vi "AlliGator Intensity Time Trace Panel.vi"() -> ()   [LabVIEW 2021, in "AlliGator Intensity Time Trace.lvlib"]
uses:
  AlliGator Intensity Time Trace.lvlib
  Globals, Variables, Constants/AlliGator Refnums List.ctl
  AlliGator Intensity Time Trace Ctrl Refnums.ctl
  Settings/AlliGator Settings List.ctl
  Action Engine/AlliGator Q Element.ctl
  Action Engine/AlliGator Q Event.ctl
  Graphs/XY Graph/XY Graph Event.ctl
  <vilib>/Utility/miscctls.llb/LVPoint32TypeDef.ctl
  Variant/Variant to Data/Variant to Boolean.vi
  Settings/AlliGator Settings+.lvlib
  Variant/Variant to Data/Variant to Data.lvlib
  Notebook/Notebook.lvlib
  Action Engine/AlliGator Action Engine.lvlib
  GUI/GUI.lvlib
  GUI/AlliGator GUI.lvlib
  Error/Error.lvlib
  Graphs/XY Graph/XY Graph Add-Ons.lvlib
  Python Plugins API/AlliGator Python Plugins.lvlib
  Decay Analysis/Decay Processing/AlliGator Decay Processing.lvlib
  Utilities/Utilities.lvlib
panel:
  in  "Use File Timestamp":bool=TRUE
  in  "Time Step":dbl[unit]=1.0 format="%#_5g"
  in  "Pin Button":bool=TRUE
  out "Intensity Time Trace TipStrip":string caption="Lifetime Graph TipStrip"
  out "Intensity Time Trace":cluster{"X Array":dbl[], "Y Array":dbl[]}[](graph)
  in  "Intensity Correction File":path
  in  "Use Intensity Correction File":bool
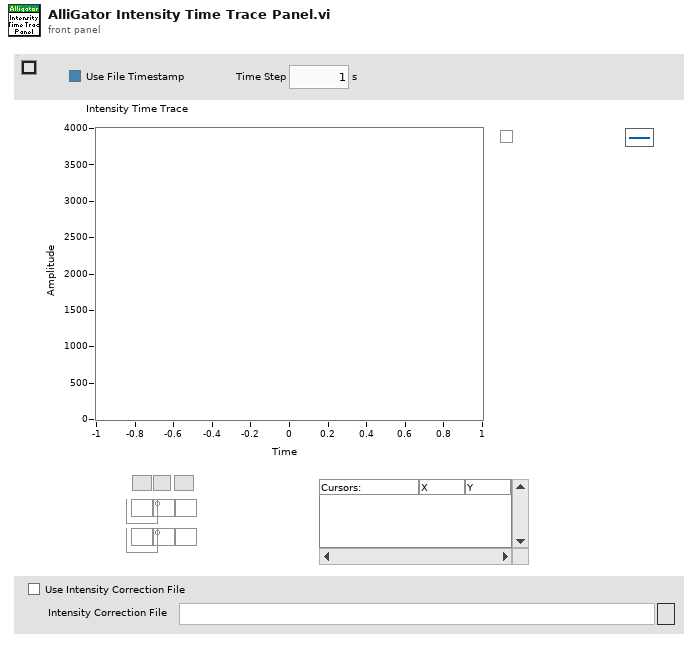
[diagram p1: front panel]
types:
  T1 = typedef "AlliGator Intensity Time Trace.lvlib/AlliGator Intensity Time Trace Ctrl Refnums.ctl" = cluster{"Intensity Time Trace":refnum<vi>, "Time Step":refnum<vi>, "Use File Timestamp":refnum<vi>}
  T2 = typedef "AlliGator GUI.lvlib/AlliGator Refnums List.ctl" = enum16{"---------- AlliGator Control Refnums ----------", "AlliGator Tab Control Refnum", "Dataset Ctrl Refnums", "Image Histogram Ctrl Refnums", "Intensity Time Trace Ctrl Refnums", "Decay Graph Ctrl Refnums", "Decay Statistics Graph Ctrl Refnums", "Phasor Graph Ctrl Refnums", "Phasor Ratio Graph Ctrl Refnums", "Phasor Plot Ctrl Refnums", "Lifetime & Other Parameters Ctrl Refnums", "Decay Fit Parameter Map Ctrl Refnums", "Parameter Map Ctrl Refnums", "Other AlliGator Ctrl Refnums", "---------- AlliGator Menu Refnums ----------", "AlliGator Menu", "---------- IO Device ID ----------", "Mouse ID", "Keyboard ID"}
  T3 = cluster{"Event Registration Refnum":refnum<event-registration>, "Event Registration Refnum":refnum<event-registration>}
  T4 = typedef "AlliGator Settings+.lvlib/AlliGator Settings List.ctl" = enum16{"GUI:Visible Settings Tab", "GUI:Last Run Version", "Source Image:Use Image Histogram for Contrast", "Source Image:Low Count Pixels Rejection Options", "Source Image:High Count Pixels Rejection Options", "Source Image:Use Image Brightness", "Source Image:Blend Overlay with Image Background", "Source Image:Use Fixed ROI Diameter", "Source Image:ROI Diameter", "Source Image:ROI Center Color", "Source Image:Peak Threshold", "Source Image:Intensity Threshold", "Source Image:Image Binning Options", "Source Image:Image Smoothing Options", "Source Image:Image Histogram Active", "Source Image:Invert Binary Mask", "Source Image:Hot Pixel Removal", "Source Image:Overlay Analyzed ROI Center", "Source Image:Auto-Adjust Contrast", "Source Image:Histogram Lower Percentile", "Source Image:Histogram Upper Percentile", "Source Image:Lock ROI with Maps", "Source Image:Save Source Image", "Source Image:Scale Bar Options", "Source Image:Image Resolution (Pixel Size)", "Source Image:Flatfield Correction", "Source Image:Show Dead Left Columns Correction", "Source Image:Dead Left Columns Correction", "Source Image:Image Pre-Processing Operations Order", "Source Image:Overlay ROI Median", "Source Image:Median Overlay Color", "Data Information:Gate Width", "Data Information:Nanotime Gate Separation", "Data Information:Macrotime Gate Separation", "Data Information:Gate Step", "Data Information:# Gates", "Data Information:Gate Image Exposure", "Data Information:Gate Image Integration", "Data Information:Gates to Skip", "Data Information:Gates to Keep", "Data Information:Define Gates to", "Data Information:Channel Name", "Data Information:Available Channel Names", "Data Information:Channel Arithmetic", "Data Information:Background File Subtraction", "Data Information:Background File", "Data Information:Background Scaling Factor", "Data Information:Background Pile-up Correction", "Data Information:Background Pixel Well Capacity", "Data Information:Laser Period", "Data Information:SYNC Period", "Data Information:Pile-up Correction", "Data Information:Pixel Well Capacity", "Data Information:Dataset Scaling Factor", "Fluorescence Decay_Decay Pre-Processing:Reverse Gates", "Fluorescence Decay_Decay Pre-Processing:Verbose Decay Pre-Processing", "Fluorescence Decay_Decay Pre-Processing:Use Decay Pre-Processing", "Fluorescence Decay_Decay Pre-Processing:Background Subtraction", "Fluorescence Decay_Decay Pre-Processing:Background Definition Range", "Fluorescence Decay_Decay Pre-Processing:Baseline Subtraction Method", "Fluorescence Decay_Decay Pre-Processing:Decay Pre-Processing Operations Order", "Fluorescence Decay_Decay Pre-Processing:Smoothing Parameter", "Fluorescence Decay_Decay Pre-Processing:Shift Decay", "Fluorescence Decay_Decay Pre-Processing:Decay Shift Parameters", "Fluorescence Decay_Decay Pre-Processing:Fold Decay", "Fluorescence Decay_Decay Pre-Processing:# Folds", "Fluorescence Decay_Decay Pre-Processing:1-Normalize Decay", "Fluorescence Decay_Decay Pre-Processing:[0-1]-Normalize Decay", "Fluorescence Decay_Decay Pre-Processing:Smoothen Decay", "Fluorescence Decay_Decay Pre-Processing:Extrapolate Decay", "Fluorescence Decay_Decay Pre-Processing:Use Periodicity", "Fluorescence Decay_Decay Pre-Processing:Use Cursors", "Fluorescence Decay_Decay Pre-Processing:Tail Fraction", "Fluorescence Decay_Decay Pre-Processing:Head Fraction", "Fluorescence Decay_Decay Pre-Processing:Additional Points", "Fluorescence Decay_Decay Pre-Processing:Straighten Decay", "Fluorescence Decay_Decay Pre-Processing:Constant Background", "Fluorescence Decay_Decay Pre-Processing:Pixel-Normalize Decay", "Fluorescence Decay_Advanced Analysis:Extract IRF instead of Decay", "Fluorescence Decay_Advanced Analysis:IRF Extraction Options", "Fluorescence Decay_Advanced Analysis:IRF Optimization Options", "Fluorescence Decay_Advanced Analysis:Square Pulse Options", "Fluorescence Decay_Advanced Analysis:IRF Order", "Fluorescence Decay_Advanced Analysis:IRF Time Constants", "Fluorescence Decay_Advanced Analysis:Wavelet Analysis Options", "Fluorescence Decay_Advanced Analysis:Average Lifetime Options", "Fluorescence Decay_Fit Options:Fit Options", "Fluorescence Decay_Fit Options:Use Legacy Fitting Approach", "Fluorescence Decay_Fit Options:Use Data Information Laser Period", "Fluorescence Decay_Fit Parameters:Displayed Fit Parameters", "Fluorescence Decay_Fit Parameters:Fit Parameter Constraints", "Fluorescence Decay_Fit Parameters:Export Tabulated Results", "Fluorescence Decay_Fit Parameters:MLE Baseline Offset Type", "Fluorescence Decay_Fit Parameters:MLE Baseline Offset", "Fluorescence Decay_Fit Parameters:Guess Parameter Names", "Fluorescence Decay_Fit Parameters:Guess Parameter Values", "Fluorescence Decay_Fit Parameters:Guess Parameters Options", "Fluorescence Decay_Fit Parameters:Optimal Offset Selection Criterion", "Fluorescence Decay_Styles:Show Last Decay Only", "Fluorescence Decay_Styles:Decay Graph Color Array", "Fluorescence Decay:Decay Graph Active", "Fluorescence Decay Statistics:Min Peak Value", "Fluorescence Decay Statistics:Reject Low Decay Peak Pixels", "Fluorescence Decay Statistics:Reject High Decay Peak Pixels", "Fluorescence Decay Statistics:Max Peak Value", "Time Traces:Use File Timestamp", "Time Traces:Time Step", "Time Traces:Use Intensity Correction File", "Time Traces:Intensity Correction File", "Phasor Plot:Phasor Plot Smoothing Options", "Phasor Plot:Phasor Plot Size", "Phasor Plot:Phasor Plot Graphics Options", "Phasor Plot:Cumulative Phasor Plot", "Phasor Plot:Use Phasor Brightness", "Phasor Plot:Blend Overlay with Phasor Background", "Phasor Plot:Save Phasor Plot", "Phasor Plot:Show References", "Phasor Plot:Phasor Ratio Decay Range", "Phasor Plot:Exponential Fading", "Phasor Plot:Phasor Ratio Reference Colors", "Phasor Plot:Reference Radius", "Phasor Plot:Show Color Map Vertices", "Phasor Plot:Phasor Plot Active", "Phasor Plot:Phasor Ratio Color Map Type", "Phasor Plot:Phasor Ratio Color Map", "Phasor Plot:Phasor Ratio Display Range", "Phasor Plot:Selected Image ROI(s)", "Phasor Plot:All Image ROIs", "Phasor Plot:Selected Phasor Plot ROI(s)", "Phasor Plot:All Phasor Plot ROIs", "Phasor Plot:Phasor Ratio Color-Coded Quantity", "Phasor Plot:Store Phasor Harmonics", "Phasor Plot:Draw Reference Segment", "Phasor Plot:User-Defined Quantity", "Phasor Plot:Color Scale High Color", "Phasor Plot:Color Scale Low Color", "Phasor Plot:Intensity-weighted Phasor Plot", "Phasor Graph:Phasor Frequency", "Phasor Graph:Phasor Ratio Type", "Phasor Graph:Pixel-level Phasor Computation", "Phasor Graph:Save Phasor Graph", "Phasor Graph:Phasor Graph Active", "Phasor Graph:Phasor SDV Options", "Phasor Graph:Intensity-weighted Phasor Graph", "Phasor Graph:Define Shortest Lifetime as", "Phasor Calibration:Use Backup Calibration if needed", "Phasor Calibration:Backup Calibration Type", "Phasor Calibration:Calibration Type", "Phasor Calibration:Calibration Lifetime", "Phasor Calibration:Calibration Map Algorithm", "Single-Exponential Phasor Locus (SEPL):Gate Parameters", "Single-Exponential Phasor Locus (SEPL):User-defined Gate", "Single-Exponential Phasor Locus (SEPL):User-defined IRF", "Single-Exponential Phasor Locus (SEPL):Phasor Parameters", "Single-Exponential Phasor Locus (SEPL):Decay & IRF Parameters", "Single-Exponential Phasor Locus (SEPL):Display Parameters", "Lifetime Analysis:Decay Analysis Parameters", "Lifetime Analysis:Lifetime Map Active", "Plugins:Python Settings", "Miscellaneous:Verbose Mode", "Miscellaneous:Beep after Script", "Miscellaneous:Saved Image File Format", "Miscellaneous:Exported Gate Image Settings", "Miscellaneous:Include Loading in Timing", "Miscellaneous:Verbose Settings Mode", "Miscellaneous:Histogram Options", "Miscellaneous:Beep on Error", "Miscellaneous:# Logical Processors Used", "Miscellaneous:ROI Description Max Characters", "Miscellaneous:Verbose Error Mode", "Miscellaneous:Transparent Mask Color"}
  T5 = typedef "AlliGator Action Engine.lvlib/AlliGator Q Element.ctl" = cluster{"AlliGator Q Event":T6, "Data":variant}
  T6 = typedef "AlliGator Action Engine.lvlib/AlliGator Q Event.ctl" = enum16{"---- Files ----", "Files:Set Batch Export Files To Save", "Files:Set Dataset Loading & Pre-processing Options", "Files:Check #Frames in Dataset", "Files:Increment Frame Index", "Files:Open Mask Image", "Files:Open White Light Image", "Files:Open Single Dataset", "Files:New Folder of Folders Selected", "Files:Load File (all Types)_Scriptable", "Files:Move Flattened Series to Folders Series", "Files:Select Folder", "Files:Load FLI Dataset", "Files:Load Swiss SPAD 1 Dataset", "Files:Load Swiss SPAD 2 Dataset", "Files:Load .sdt FLI Dataset", "Files:Load .ptu FLI Dataset", "Files:Load .bin FLI Dataset", "Files:Load Single Gate Image Folder", "Files:Load I/m/phi Dataset (deprecated)", "Files:Load Single Image", "Files:Subtract Background File", "Files:Export FLI Dataset", "Files:Load HDF5 FLI Dataset", "Files:Set Destination File Path", "Files:Save Mask Image", "Files:Batch Conversion", "Files:New Folder Selected", "Files:Close FLI Dataset", "Files:Close FLI Dataset Series", "Files:Close White Light Image", "Files:Close Mask Image", "---- FLI Dataset ----", "FLI Dataset:Channel Arithmetic", "FLI Dataset:Export Average Lifetime Map as ASCII", "FLI Dataset:Export User-Defined Quantity Map as ASCII", "FLI Dataset:Python Function FLI Dataset Event", "FLI Dataset:ROI Analysis", "FLI Dataset:Tilted Logistic Square Gated IRF Characteristics Map", "FLI Dataset:Logistic Square Gated IRF Characteristics Map", "FLI Dataset:Square Gated IRF Characteristics Map", "FLI Dataset:Multi-ROI Single-Pixel Phasor Analysis", "FLI Dataset:Multi-ROI Single-Pixel NLSF Analysis", "FLI Dataset:All ROIs IRF Extraction", "FLI Dataset:All ROIs Decay Fit Non-Interactive (Fast + Individual IRF)", "FLI Dataset:All ROIs Phasor Analysis", "FLI Dataset:All ROIs Decay Fit", "FLI Dataset:Fluorescence Decay Statistics", "FLI Dataset:Update Decay Statistics Graph", "FLI Dataset:Get Decay from ROI", "FLI Dataset:All ROIs Average Lifetimes", "FLI Dataset:Save/Load Local IRFs", "FLI Dataset:Clear Local IRFs", "FLI Dataset:Phasor Calibration Maps (# Gates Series) Script", "FLI Dataset:Calibrated Phasor Map Series", "---- FLI Dataset Series ----", "FLI Dataset Series:Sum All Datasets in Series", "FLI Dataset Series:Add Dataset to Accumulated Dataset", "FLI Dataset Series:Display Accumulated Dataset", "FLI Dataset Series:Clear Dataset Series Sum", "FLI Dataset Series:Time-Series Analysis (NLSF)", "FLI Dataset Series:Time-Series Analysis (Phasor)", "---- Image ----", "Image:Update Image Profile Plots", "Image:Image Histogram Cursor Move", "Image:Image Histogram", "Image:Image Contrast", "Image:Set Image Histogram Cursor Move Flag", "Image:Clear Image Overlay", "Image:Use ROI as Search Area", "Image:Set ROI Diameter", "Image:Save Image Data as TIFF", "Image:Save Displayed Image with Overlay", "Image:Save Image Overlay Only", "Image:Save Image as Hot Pixel Mask", "Image:Change Source Image Color Palette", "Image:Copy Image to Clipboard", "Image:Source Image ROI Selection", "Image:Delete All ROIs", "Image:Delete All Unselected ROIs", "Image:Delete ROI", "Image:Merge All ROIs", "Image:Store ROI", "Image:Source Image ROI Storage", "Image:Export ROI Description to Notebook", "Image:Save ROI", "Image:Load ROI", "Image:Paste ROI Definition", "Image:Clear ROI", "Image:Identify ROIs in Mask Image", "Image:Create Complementary ROI", "Image:Create Contour ROI", "Image:Create ROI(s) from Pixels with Peak above Min_Scriptable", "Image:Create ROI(s) from Pixels with Intensity above Min_Scriptable", "Image:Compute ROI Statistics", "Image:Delete ROI(s) based on ROI Characteristics", "Image:Create ROI Grid", "Image:ROI to Individual Pixel ROIs", "Image:Python Function Source Image Event", "Image:Show Phasor Calibration Map ROI Centers", "Image:Convert ROI to Mask Image", "Image:Mouse Move", "Image:Mouse Up", "Image:Set Source Image Mouse Move Flag", "Image:Add Scale Bar Overlay", "Image:Delete Existing ROIs Option", "Image:Overlay ROI Median", "Image:Check Current ROI", "Image:Update True Pixel Value", "Image:Use ROI", "---- Decay ----", "Decay:Clear IRF/Reference Plot", "Decay:Add Decay to Graph", "Decay:Smoothen Plot", "Decay:Smoothen Plot Tail", "Decay:Average Selected Plots", "Decay:Extract IRF", "Decay:Optimal IRF Extraction", "Decay:Threshold IRF", "Decay:Fit to Model IRF", "Decay:Fit IRF to Square Gate", "Decay:Fit IRF to Logistic Square Gate", "Decay:Fit IRF to Tilted Logistic Square Gate", "Decay:Create Bounding Cursors Set", "Decay:Export Bounding Cursors Definition to Notebook", "Decay:Denoise Plot", "Decay:Compute Cumulative Function", "Decay:Use as Reference Decay", "Decay:Show Reference Decay/IRF", "Decay:Extrapolate Decay", "Decay:Create Head & Tail Bounding Cursors", "Decay:Store Cursor-defined Head & Tail Fractions", "Decay:Rebin Plot", "Decay:1-Normalize Decay", "Decay:[0-1]-Normalize Plot", "Decay:Straighten Decay", "Decay:Shift Decay", "Decay:Fold Decay", "Decay:Fit Decay", "Decay:Global Fit of Selected Decays", "Decay:Post Global Fit Script", "Decay:Add Global Fit Parameters to Graph", "Decay:Add Decay Parameter(s) to Plot (Graph)", "Decay:Export Decay to Phasor Graph", "Decay:Compute Average Lifetime", "Decay:Plot Convolution", "Decay:Graph Tip Strip Update", "---- Decay Statistics ----", "Decay Statistics:Tip Strip Update", "---- Intensity Time Trace ----", "Intensity Time Trace:Use File Timestamp", "Intensity Time Trace:Load Intensity Corrections File", "Intensity Time Trace:Clear Intensity Corrections File", "Intensity Time Trace:Tip Strip Update", "---- Phasor Plot ----", "Phasor Plot:Build Phasor Plot", "Phasor Plot:Change Phasor Plot Color Palette", "Phasor Plot:Adjust Phasor Plot Display Range", "Phasor Plot:Highlight Image ROI in Phasor Plot", "Phasor Plot:Save Phasor Plot Image with Overlay", "Phasor Plot:Export Complex Phasor Map", "Phasor Plot:Export Phasor Ratio Map", "Phasor Plot:Export Average Lifetime Map", "Phasor Plot:Compute Phase Lifetime Histogram", "Phasor Plot:Compute Phasor Ratio Histogram", "Phasor Plot:Compute Phase Lifetime vs Intensity Scatter Plot", "Phasor Plot:Weber 2-Component Decomposition", "Phasor Plot:Update Phasor Color Map Vertices", "Phasor Plot:Clear Phasor Overlay", "Phasor Plot:Use Segment Extremities as References", "Phasor Plot:Use UC/Segment Intersections as References", "Phasor Plot:Use UC/Principal Axis Intersections as References", "Phasor Plot:Use UC/Linear Fit Intersections as References", "Phasor Plot:Update Phasor Plot Reference", "Phasor Plot:Show Local Phasor Info in Phasor Plot", "Phasor Plot:Update Phasor Plot State", "Phasor Plot:Phasor Plot ROI Storage", "Phasor Plot:Phasor Plot ROI Selection", "Phasor Plot:Python Function Phasor Plot Event", "Phasor Plot:Overlay Phasor ROI, Ratio or Map in Source Image", "Phasor Plot:Compute Decay of Selected Phasors", "Phasor Plot:Phasor at Image Pixel", "Phasor Plot:Mouse Move", "Phasor Plot:Mouse Up", "Phasor Plot:Display Range Mouse Move", "Phasor Plot:Set Mouse Move Flag", "Phasor Plot:Update True Phasor Plot Value", "---- Phasor Graph ----", "Phasor Graph:Get Phasor Value", "Phasor Graph:Create New Phasor Plot Dialog", "Phasor Graph:Update Last Phasor Value", "Phasor Graph:Update Phasor (m, phi)", "Phasor Graph:Remove Single Phasor from Plot", "Phasor Graph:Add Single Phasor to Plot", "Phasor Graph:Remove Phasor Plot", "Phasor Graph:Remove Selected Phasor Plots", "Phasor Graph:Clear Phasor Data", "Phasor Graph:Clear Phasor Graph", "Phasor Graph:Cursor Move", "Phasor Graph:Draw Cursor Connecting Line", "Phasor Graph:Clear Cursor Connecting Line", "Phasor Graph:Find UC Intersection", "Phasor Graph:Use UC/Cursor-Defined Line Intersections", "Phasor Graph:Use Selected Plots Fitted Line/UC Intersections", "Phasor Graph:Use Selected Plots Principal Axis/UC Intersections", "Phasor Graph:Show Single Phasor", "Phasor Graph:Save Single Phasor Plot", "Phasor Graph:Save All Phasor Plots", "Phasor Graph:Load Phasor Plot(s)", "Phasor Graph:Phasor Multiplication", "Phasor Graph:Compute Average Phasor", "Phasor Graph:Compute Multiple Average Phasors (Selected Plots)", "Phasor Graph:Export Single Phasor Plot Phase Lifetimes", "Phasor Graph:Parameter 2 vs Parameter 1 Scatter Plot", "Phasor Graph:Use Cursor n Location", "Phasor Graph:Set Reference n to Current Phase Lifetime Value", "Phasor Graph:Set Reference n to Lifetime Value", "Phasor Graph:Set Cursor n Location", "Phasor Graph:Save Phasor Graph Image", "Phasor Graph:Update SEPL Plot", "Phasor Graph:Export Single Phasor Plot Data", "Phasor Graph:Export Selected Phasor Plots Data", "Phasor Graph:Python Function Phasor Graph Event", "Phasor Graph:Tip Strip Update", "---- Calibration ----", "Calibration:Set Calibration Type", "Calibration:Load/Save Phasor Calibration", "Calibration:Load/Save Phasor Calibration Series", "Calibration:Load/Save Phasor Calibration Map", "Calibration:Use as Calibration", "Calibration:Compute Optimal Calibration from Phasor References", "Calibration:Clear Phasor Calibration", "Calibration:Single Phasor Calibration Information", "Calibration:Use as Calibration Series", "Calibration:Use as Calibration Map", "Calibration:Clear Calibration Series", "Calibration:Phasor Calibration Series Information", "Calibration:Clear Calibration Map", "Calibration:Phasor Calibration Map Information", "Calibration:Apply Phasor Calibration", "Calibration:Update Single Plot Calibration", "Calibration:Update Multiple Plots Calibration", "Calibration:Clear Single Plot Calibration", "Calibration:Clear All Plots Calibrations", "Calibration:Clear Plot(s) Calibration(s)?", "---- Phasor Ratio ----", "Phasor Ratio:Clear Reference n", "Phasor Ratio:Toggle Selected Plot(s)  Lock to Reference 1", "Phasor Ratio:Use as Reference n", "Phasor Ratio:Send Reference n to Notebook", "Phasor Ratio:Toggle Selected Plot(s)  Lock to Reference 2", "Phasor Ratio:Compute Phasor Ratio at Mouse Location", "Phasor Ratio:Compute Phasor Plot's Average Phasor Ratio", "Phasor Ratio:Compute Time-Series Phasor Ratios", "Phasor Ratio:Fit Line to Phasor Ratio Plot", "Phasor Ratio:Save References", "Phasor Ratio:Load References", "Phasor Ratio:Update Phasor Reference 1", "Phasor Ratio:Update Phasor Reference 2", "Phasor Ratio:Move Cursor n to Reference n", "Phasor Ratio:Use as Phasor Reference 1 Lifetime", "Phasor Ratio:Use as Phasor Reference 2 Lifetime", "Phasor Ratio:Export Phasor Ratio Map as ASCII", "Phasor Ratio:Tip Strip Update", "---- Lifetime & Other Parameters Graph ----", "Lifetime:Compute Sliced Mean, SDV and CV Plots", "Lifetime:Plot Decay Shifts", "Lifetime:Plot Histogram", "---- Decay Fit Parameter Map ----", "Decay Fit Parameter Map:Export ROI NLSF Data as ASCII", "Decay Fit Parameter Map:Set Decay Fit Parameter Map Selection", "Decay Fit Parameter Map:Build Decay Fit Parameter Map", "Decay Fit Parameter Map:Change Decay Fit Parameter Map Color Palette", "Decay Fit Parameter Map:Export Decay Fit Parameter Map Data as ASCII", "Decay Fit Parameter Map:Export All Decay Fit Parameter Maps Data as ASCII", "Decay Fit Parameter Map:Selected Parameter Scatterplot", "Decay Fit Parameter Map:Parameter 2 vs Parameter 1 Scatterplot", "Decay Fit Parameter Map:Save Decay Fit Parameter Map Image", "Decay Fit Parameter Map:Save-Load IRFs & Fit Data", "Decay Fit Parameter Map:Update Local Decay Plots", "Decay Fit Parameter Map:Python Function Decay Fit Parameters Map Event", "Decay Fit Parameter Map:Overlay Decay Fit Parameter Map in Source Image", "Decay Fit Parameter Map:Selected Parameter vs Intensity Scatterplot", "Decay Fit Parameter Map:Mouse Up", "Decay Fit Parameter Map:Mouse Move", "Decay Fit Parameter Map:Display Range Mouse Move", "Decay Fit Parameter Map:Change Map Resolution", "Decay Fit Parameter Map:Variance Significance Maps", "Decay Fit Parameter Map:Fit Result Constraints Window", "Decay Fit Parameter Map:Use ROI", "---- Parameter Map ----", "Parameter Map:Export ROI Parameters Data as ASCII", "Parameter Map:Add Parameter Map Set", "Parameter Map:Delete Parameter Map Set", "Parameter Map:Update Parameter List", "Parameter Map:Build Parameter Map", "Parameter Map:Change Parameter Map Color Palette", "Parameter Map:Export Parameter Map Data as ASCII", "Parameter Map:Export All Parameter Maps Data as ASCII", "Parameter Map:Selected Parameter Scatterplot", "Parameter Map:Parameter 2 vs Parameter 1 Scatterplot", "Parameter Map:Selected Parameter vs Intensity Scatterplot", "Parameter Map:Save Parameter Map Image", "Parameter Map:Save-Load IRFs & Parameter Maps (TODO)", "Parameter Map:Set Parameter Map Selection", "Parameter Map:Python Function Parameter Map Event", "Parameter Map:Overlay Parameter Map in Source Image", "Parameter Map:Update Local Decay Plots", "Parameter Map:Mouse Up", "Parameter Map:Mouse Move", "Parameter Map:Display Range Mouse Move", "Parameter Map:Use ROI", "---- Generic Graph ----", "Generic Graph:Generic XY Graph Event", "Generic Graph:Python Function XY Graph Event", "Generic Graph:New Plot", "Generic Graph:Save Plot", "Generic Graph:XY Plot Histogram", "Generic Graph:Set XY Graph Plot Name", "Generic Graph:Set Last Cursor Style", "Generic Graph:Tip Strip Update", "---- GUI ----", "GUI:Start Script", "GUI:Type of Displayed Image Changed", "GUI:Gate Image Slide Changed", "GUI:Show Busy Icon", "GUI:Show Busy Icon & Abort Button", "GUI:Hide Busy Icon", "GUI:Hide Busy Icon & Abort Button", "GUI:Abort", "GUI:End Script", "GUI:Start Timing", "GUI:End Timing", "GUI:Set State Indicator", "GUI:Send Parameters JSON Strings to Clipboard", "GUI:Set Gate Step", "GUI:Idle", "GUI:Initialization", "GUI:Quit", "GUI:Increment Dataset Index", "GUI:Set Dataset Index to -1", "GUI:Time Series Slider Moved", "GUI:Time Series Slider Changed", "GUI:Toggle Playback or Loop", "GUI:Playback Script", "GUI:Set Phasor Frequency", "GUI:Open Window", "GUI:Start Test Script", "GUI:End Test Script", "GUI:Set Verbose Mode", "GUI:Set Verbose Settings Mode", "GUI:Initialize Python Session", "DEBUG"}
  T7 = typedef "XY Graph Add-Ons.lvlib/XY Graph Event.ctl" = cluster{"Item Tag":string, "XY Graph Refnum":refnum<vi>, "Coords":T8, "Item Path":string}
  T8 = typedef "LVPoint32TypeDef.ctl" = cluster{"Horizontal":i32, "Vertical":i32}
  T9 = enum16{"0", "1", "2", "3", "4", "5", "6", "7", "8", "9", "A", "B", "C", "D", "E", "F", "G", "H", "I", "J", "K", "L", "M", "N", "O", "P", "Q", "R", "S", "T", "U", "V", "W", "X", "Y", "Z", "F1", "F2", "F3", "F4", "F5", "F6", "F7", "F8", "F9", "F10", "F11", "F12", "F13", "F14", "F15", "ADD", "BACK", "BACKSLASH", "CAPITAL", "COMMA", "DECIMAL", "DELETE", "DIVIDE", "DOWN", "END", "EQUALS", "ESCAPE", "GRAVE (`)", "HOME", "INSERT", "LBRACKET", "LCONTROL", "LEFT", "L ALT", "LSHIFT", "LWIN", "MINUS", "MULTIPLY", "NEXT", "NUMLOCK", "NUMPAD_0", "NUMPAD_1", "NUMPAD_2", "NUMPAD_3", "NUMPAD_4", "NUMPAD_5", "NUMPAD_6", "NUMPAD_7", "NUMPAD_8", "NUMPAD_9", "PAUSE", "PERIOD", "PRIOR (PG UP)", "RBRACKET", "RCONTROL", "RETURN", "RIGHT", "R ALT", "RSHIFT", "RWIN", "SCROLL", "SEMICOLON", "SLASH", "SPACE", "SUBTRACT", "TAB", "UP", "ENTER (num pad)", "' (quote)"}
  T10 = enum16{"0", "1", "2", "3", "4", "5", "6", "7", "8", "9", "A", "B", "C", "D", "E", "F", "G", "H", "I", "J", "K", "L", "M", "N", "O", "P", "Q", "R", "S", "T", "U", "V", "W", "X", "Y", "Z", "F1", "F2", "F3", "F4", "F5", "F6", "F7", "F8", "F9", "F10", "F11", "F12", "F13", "F14", "F15", "ADD", "BACK", "BACKSLASH", "CAPITAL", "COMMA", "DECIMAL", "DELETE", "DIVIDE", "DOWN", "END", "EQUALS", "ESCAPE", "GRAVE (`)", "HOME", "INSERT", "LBRACKET", "LCONTROL", "LEFT", "L ALT", "LSHIFT", "LWIN", "MINUS", "MULTIPLY", "NEXT", "NUMLOCK", "NUMPAD_0", "NUMPAD_1", "NUMPAD_2", "NUMPAD_3", "NUMPAD_4", "NUMPAD_5", "NUMPAD_6", "NUMPAD_7", "NUMPAD_8", "NUMPAD_9", "PAUSE", "PERIOD", "PRIOR (PG UP)", "RBRACKET", "RCONTROL", "RETURN", "RIGHT", "R ALT", "RSHIFT", "RWIN", "SCROLL", "SEMICOLON", "SLASH", "SPACE", "SUBTRACT", "TAB", "UP", "ENTER (num pad)", "' (quote)"}[]
  T11 = typedef "XY Graph Add-Ons.lvlib/XY Graph Refnum.ctl" = refnum<vi>
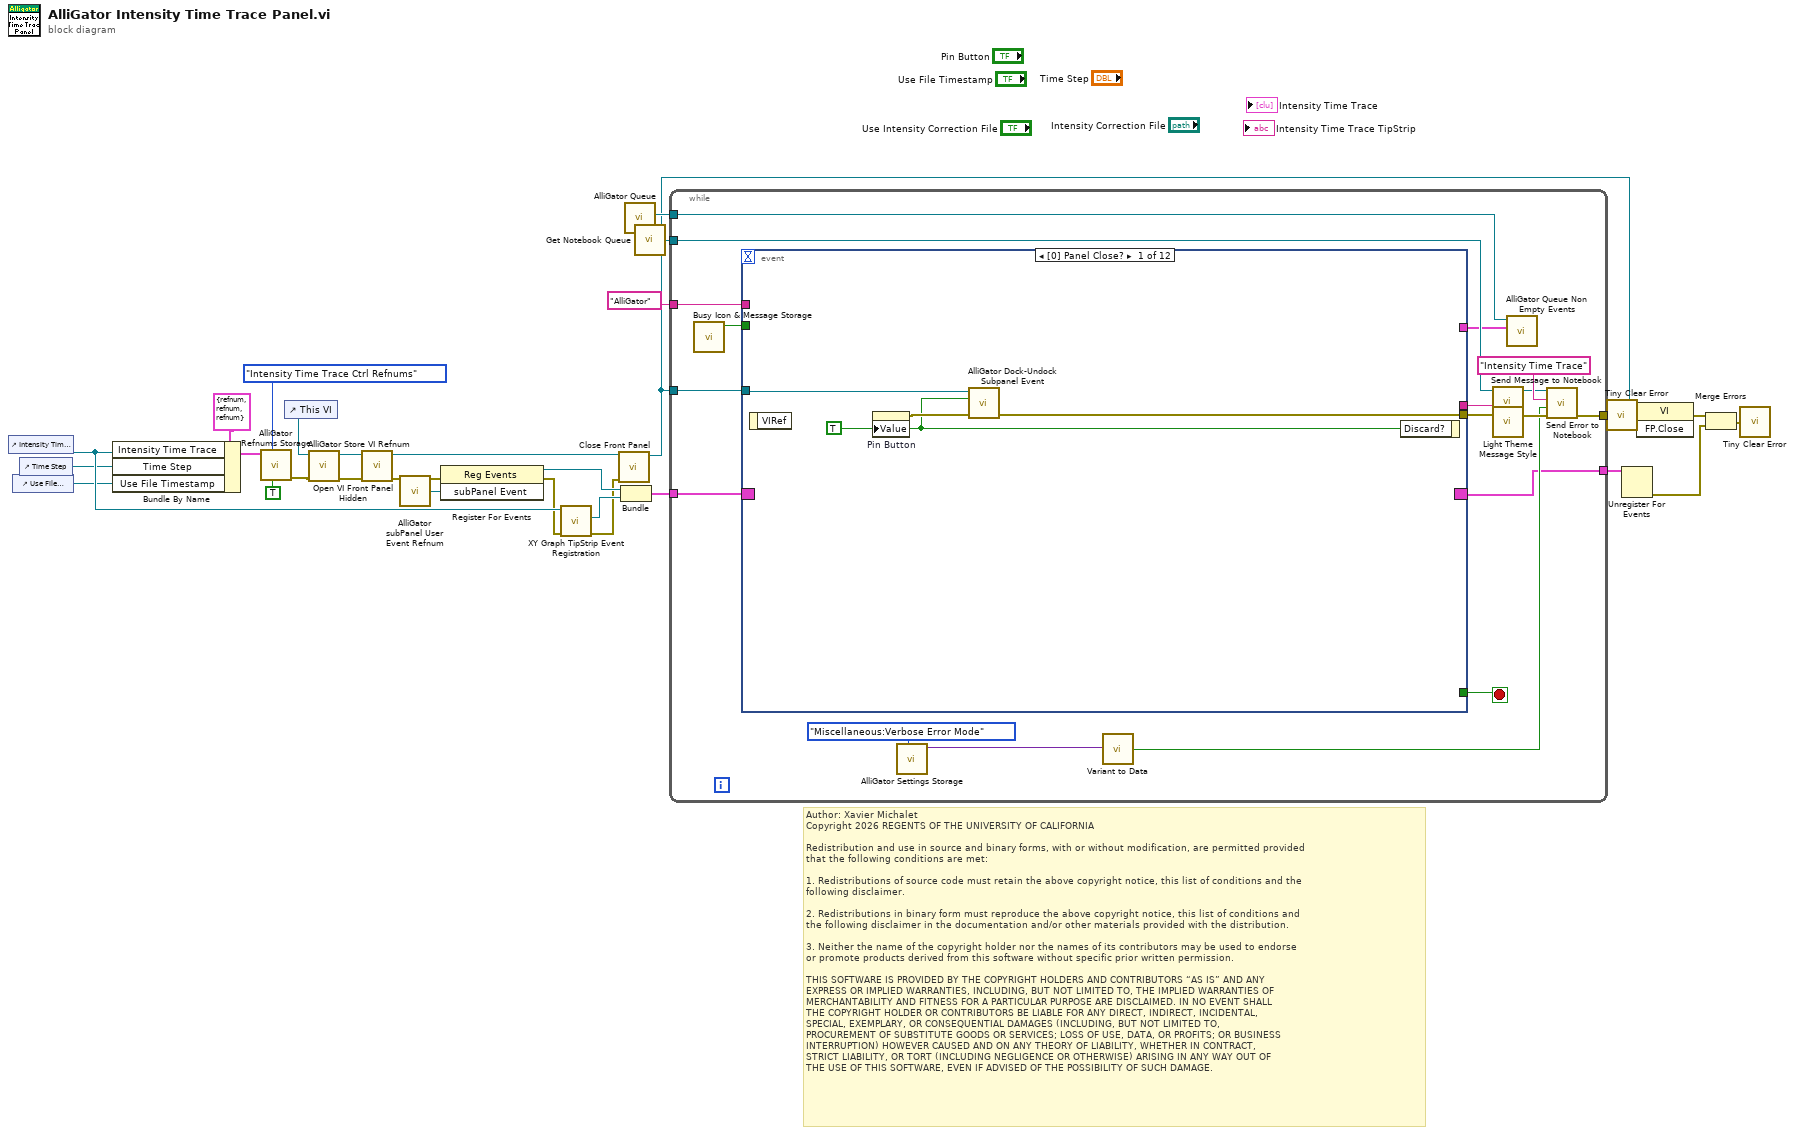
[diagram p0: block diagram]
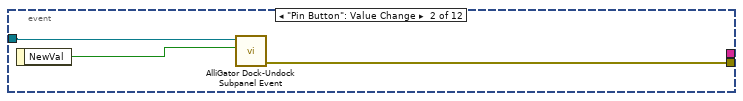
[diagram p2: hidden frame]
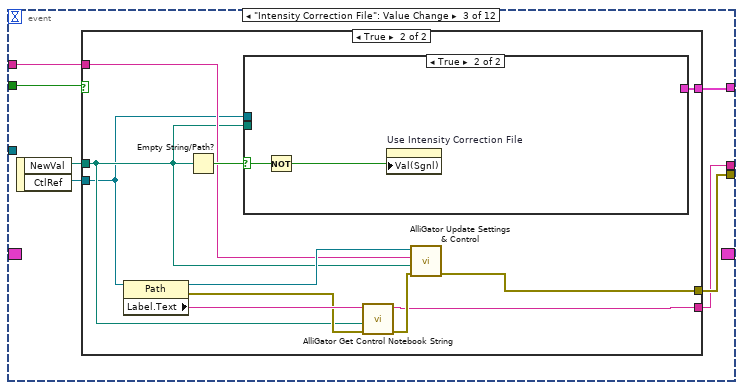
[diagram p3: hidden frame]
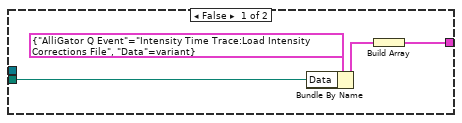
[diagram p5: hidden frame]
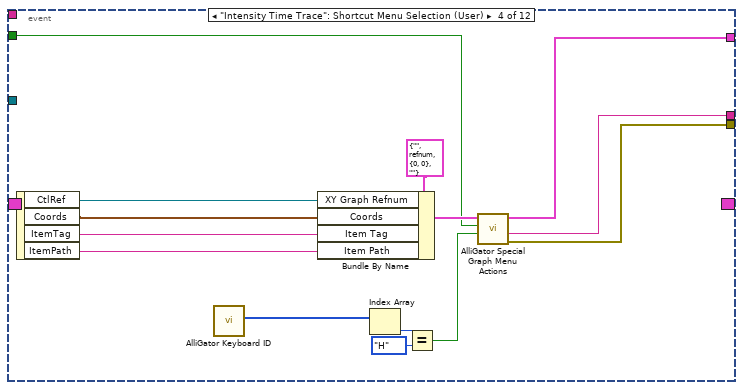
[diagram p6: hidden frame]
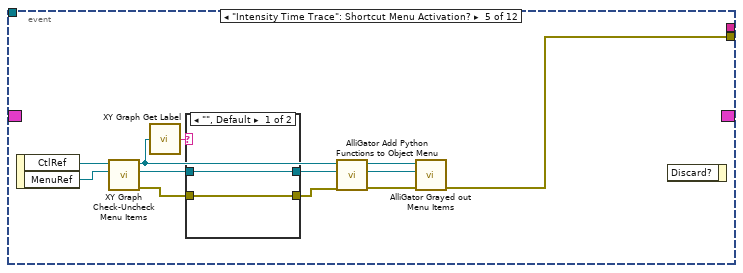
[diagram p7: hidden frame]
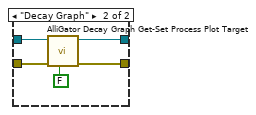
[diagram p8: hidden frame]
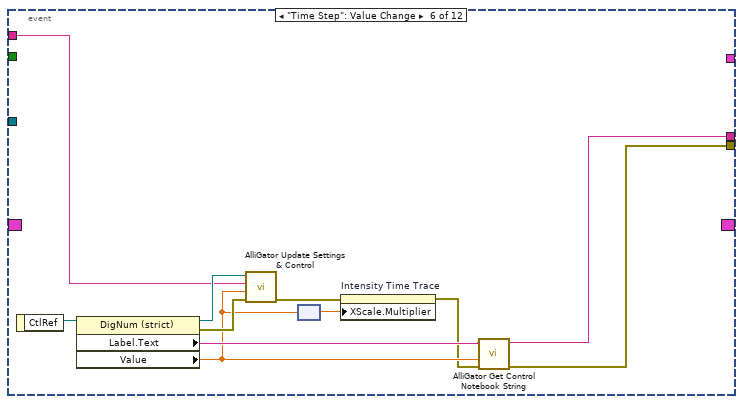
[diagram p9: hidden frame]
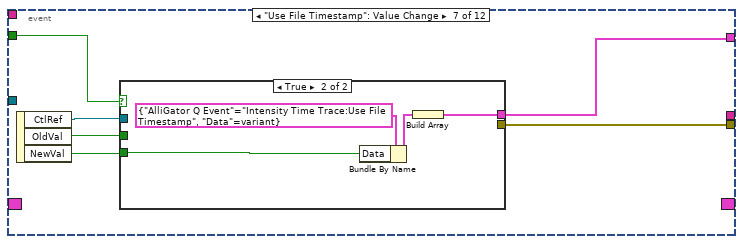
[diagram p10: hidden frame]
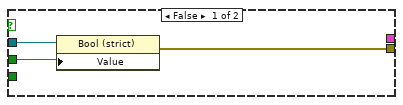
[diagram p11: hidden frame]
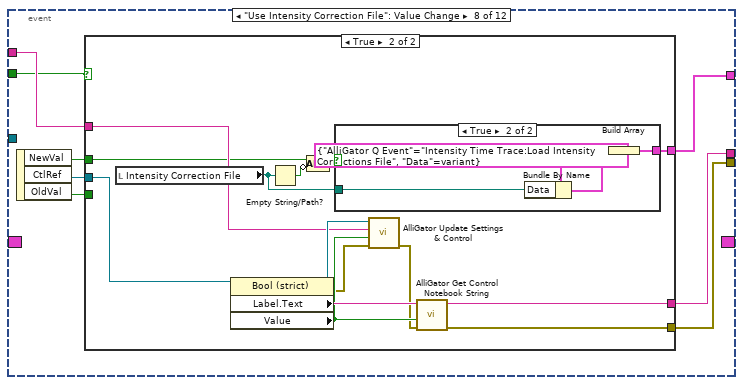
[diagram p12: hidden frame]
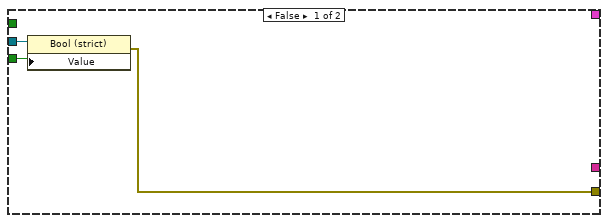
[diagram p13: hidden frame]
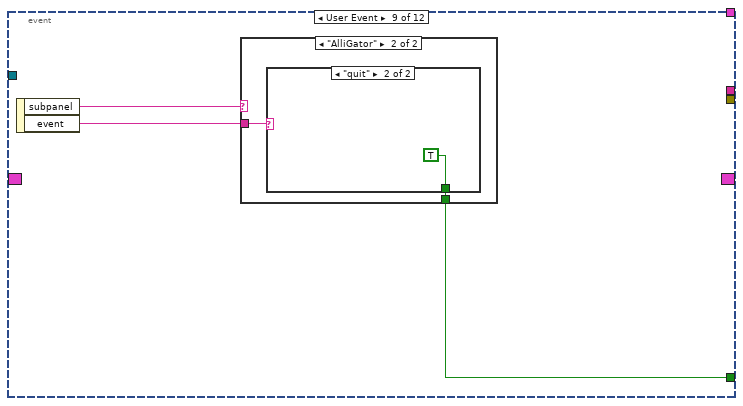
[diagram p15: hidden frame]
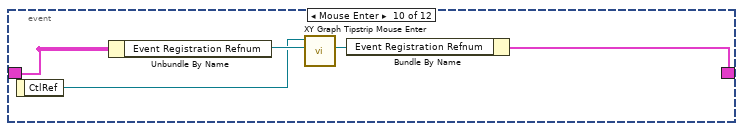
[diagram p18: hidden frame]
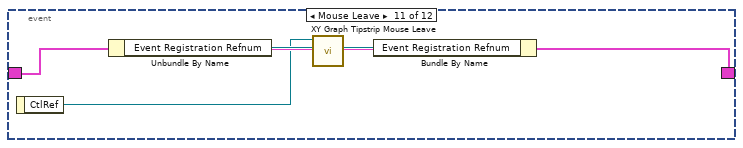
[diagram p19: hidden frame]
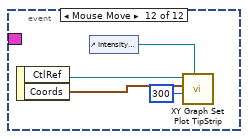
[diagram p20: hidden frame]
diagram:
  # "Author: Xavier Michalet\nCopyright 2026 REGENTS OF THE UNIVERSITY OF CALIFORNIA\n\nRedistribution and use in source and binary forms, with or without modification, are permitted provided\nthat the following conditions are met:\n\n1. Redistributions of source code must retain the above copyright notice, this list of conditions and the\nfollowing disclaimer.\n\n2. Redistributions in binary form must reproduce the above copyright notice, this list of conditions and\nthe following disclaimer in the documentation and/or other materials provided with the distribution.\n\n3. Neither the name of the copyright holder nor the names of its contributors may be used to endorse \nor promote products derived from this software without specific prior written permission.\n\nTHIS SOFTWARE IS PROVIDED BY THE COPYRIGHT HOLDERS AND CONTRIBUTORS “AS IS” AND ANY \nEXPRESS OR IMPLIED WARRANTIES, INCLUDING, BUT NOT LIMITED TO, THE IMPLIED WARRANTIES OF\nMERCHANTABILITY AND FITNESS FOR A PARTICULAR PURPOSE ARE DISCLAIMED. IN NO EVENT SHALL\nTHE COPYRIGHT HOLDER OR CONTRIBUTORS BE LIABLE FOR ANY DIRECT, INDIRECT, INCIDENTAL, \nSPECIAL, EXEMPLARY, OR CONSEQUENTIAL DAMAGES (INCLUDING, BUT NOT LIMITED TO, \nPROCUREMENT OF SUBSTITUTE GOODS OR SERVICES; LOSS OF USE, DATA, OR PROFITS; OR BUSINESS\nINTERRUPTION) HOWEVER CAUSED AND ON ANY THEORY OF LIABILITY, WHETHER IN CONTRACT, \nSTRICT LIABILITY, OR TORT (INCLUDING NEGLIGENCE OR OTHERWISE) ARISING IN ANY WAY OUT OF\nTHE USE OF THIS SOFTWARE, EVEN IF ADVISED OF THE POSSIBILITY OF SUCH DAMAGE."
  n1 = control-ref of="Intensity Time Trace"() -> (w12:refnum<vi>)
  n2 = control-ref of="Use File Timestamp"() -> (w10:refnum<vi>)
  n3 = control-ref of="Time Step"() -> (w11:refnum<vi>)
  n4 = Bundle By Name(cluster=T1 {"Intensity Time Trace"=refnum, "Time Step"=refnum, "Use File Timestamp"=refnum} ("Intensity Time Trace Ctrl Refnums"), "Intensity Time Trace"=w12, "Time Step"=w11, "Use File Timestamp"=w10) -> (w17:T1)
  n5 = call "AlliGator Refnums Storage.vi"("Get(F)/Set"=TRUE, "AlliGator Refnum List"=AlliGator_Refnums_List."Intensity Time Trace Ctrl Refnums", "Data in"=w17) -> ("Error Out"=w2:errorcluster)  [unwired: 7 in, 1 out]
  n6 = control-ref of="This VI"() -> (w4:refnum<vi>)
  n7 = call "AlliGator Store VI Refnum.vi"("error in (no error)"=w2, "VI Refnum"=w4) -> ("error out"=w1:errorcluster, "VI Refnum (dup)"=w3:refnum<vi>)  [unwired: 7 in, 1 out]
  n8 = call "Open VI Front Panel Hidden.vi"("error in"=w1, "VI in"=w3) -> ("error out"=w9:errorcluster, "VI out"=w6:refnum<vi>)  [unwired: 8 in]
  n9 = call "AlliGator subPanel User Event Refnum.vi"() -> ("subPanel Event"=w26:refnum<user-event>)  [unwired: 9 in]
  n10 = register-events(error in=w9, w26) -> (reference out=w25:refnum<event-registration>, error out=w8:errorcluster)  [unwired: 1 in]
  n11 = call "XY Graph TipStrip Event Registration.vi"("error in (no error)"=w8, "XY Graph Refnum"=w12) -> ("error out"=w7:errorcluster, "Event Registration Refnum"=w18:refnum<event-registration>)  [unwired: 7 in, 1 out]
  n12 = call "Close Front Panel.vi"("error in (no error)"=w7, "VI in"=w6) -> ("VI out"=w5:refnum<vi>)  [unwired: 8 in, 1 out]
  n13 = Bundle("Event Registration Refnum"=w25, "Event Registration Refnum"=w18) -> (w19:T3)  [unwired: 1 in]
  n14 = call "AlliGator Queue.vi"() -> ("AlliGator Q"=w28:refnum<queue>)  [unwired: 8 in, 1 out]
  n15 = call "Get Notebook Queue.vi"() -> ("Notebook Queue"=w29:refnum<queue>)  [unwired: 9 in]
  n16 = while {
    tunnel: w29 -> [w40]
    tunnel: w28 -> [w37]
    tunnel: "AlliGator" ("Sender") -> [w35]
    tunnel: w5 -> [w33]
    tunnel: w19 -> [w32]
    tunnel: [w31] -> w24
    tunnel: [w30] -> w23
    stop <- w47 stop-if-true
    n17 = call "Busy Icon & Message Storage.vi"() -> ("Busy Icon Status (F = busy)"=w34:bool)  [unwired: 9 in, 2 out]
    n18 = event shown="[0] Panel Close?" {
      selector: w32 -> [_ _ _ _ _ _ _ _ _ w173 w178 _]
      dyn-events: [_ _ _ _ _ _ _ _ _ w171 w176 _] -> w31
      timeout: _ -> [_ _ _ _ _ _ _ _ _ _ _ _]
      tunnel: [w50 w54 w57 w79 w93 w115 w123 w136 _ _ _ _] -> w41
      tunnel: [_ _ _ _ _ _ _ _ w165 _ _ _] -> w47
      tunnel: [_ _ w56 w80 _ w116 _ w137 _ _ _ _] -> w38
      tunnel: [_ _ w58 w81 _ _ w124 w138 _ _ _ _] -> w36
      tunnel: w34 -> [_ _ w55 w82 _ _ w125 w139 _ _ _ _]
      tunnel: w35 -> [_ _ w59 _ _ w119 _ w140 _ _ _ _]
      tunnel: w33 -> [w49 w53 _ _ _ _ _ _ _ _ _ _]
      event Panel Close? {
        w48 = TRUE ("Pin Button")
        n19 = event-data() -> ()  [unwired: 1 in, 1 out]
        n20 = property on="Pin Button" class="Bool (strict)"("Value"=w48) -> (error out=w51:errorcluster)  [unwired: 2 in, 1 out]
        n21 = call "AlliGator Dock-Undock Subpanel Event.vi"("Error In"=w51, "Dock?"=w48, "VI in"=w49) -> ("Error Out"=w50:errorcluster)  [unwired: 8 in]
        n22 = event-data("Discard?"=w48) -> ()  [unwired: 1 in, 1 out]
      }
      event "Pin Button": Value Change {
        n23 = event-data() -> ("NewVal"=w52:bool)  [unwired: 1 in]
        n24 = call "AlliGator Dock-Undock Subpanel Event.vi"("Dock?"=w52, "VI in"=w53) -> ("Error Out"=w54:errorcluster)  [unwired: 9 in]
      }
      event "Intensity Correction File": Value Change {
        n25 = event-data() -> ("NewVal"=w61:path, "CtlRef"=w60:refnum<vi>)  [unwired: 1 in]
        n26 = case shown="True" w55 {
          tunnel: w61 -> [_ w65]
          tunnel: w59 -> [_ w69]
          tunnel: w60 -> [_ w62]
          tunnel: [_ w66] -> w57
          tunnel: [_ w64] -> w58
          tunnel: [_ w63] -> w56
          frame False {
          }
          frame True {
            n27 = property class="Path"(reference=w62) -> (reference out=w70:refnum<vi>, error out=w68:errorcluster, "Label.Text"=w71:string)  [unwired: 1 in]
            n28 = Empty String/Path?(string/path=w65) -> (empty?=w72:bool)
            n29 = case shown="True" w72 {
              selector: w72 -> [_ w78]
              tunnel: w65 -> [w74 _]
              tunnel: [w73 _] -> w64
              tunnel: w62 -> [_ _]
              frame False {
                n30 = Bundle By Name(cluster=T5 {"AlliGator Q Event"=enum."Intensity Time Trace:Load Intensity Corrections File", "Data"=variant} ("Time-Gated Phasor Q Element"), "Data"=w74) -> (w75:T5)
                n31 = Build Array(w75) -> (w73:T5[])
              }
              frame True {
                n32 = Not(x=w78) -> (.not. x?=w77:bool)
                n33 = property on="Use Intensity Correction File" class="Bool (strict)"("Val(Sgnl)"=w77) -> ()  [unwired: 2 in, 2 out]
              }
            }
            n34 = call "AlliGator Get Control Notebook String.vi"("error in (no error)"=w68, "Value"=w65, "Control Label"=w71) -> ("error out"=w67:errorcluster, "Notebook String"=w63:string)  [unwired: 7 in]
            n35 = call "AlliGator Update Settings & Control.vi"("Error In"=w67, "Value"=w65, "Sender"=w69, "CtlRef"=w70) -> ("Error Out"=w66:errorcluster)  [unwired: 7 in]
          }
        }
      }
      event "Intensity Time Trace": Shortcut Menu Selection (User) {
        n36 = event-data() -> ("CtlRef"=w86:refnum<vi>, "Coords"=w85:T8, "ItemTag"=w84:string, "ItemPath"=w83:string)  [unwired: 1 in]
        n37 = call "AlliGator Keyboard ID.vi"() -> ("keys pressed"=w87:T10)  [unwired: 9 in, 2 out]
        n38 = Bundle By Name(cluster=T7 {"Item Tag"="", "XY Graph Refnum"=refnum, "Coords"={"Horizontal"=0, "Vertical"=0}, "Item Path"=""} ("XY Graph Event"), "XY Graph Refnum"=w86, "Coords"=w85, "Item Tag"=w84, "Item Path"=w83) -> (w89:T7)
        n39 = Index Array(array=w87) -> (element=w92:T9)  [unwired: 1 in]
        n40 = Equal?(x=w92, y=T9."H" ("element")) -> (x = y?=w88:bool)
        n41 = call "AlliGator Special Graph Menu Actions.vi"("Help?"=w88, "Animated Busy Icon"=w82, "XY Graph Event"=w89) -> ("Error Out"=w79:errorcluster, "Message"=w80:string, "AlliGator Actions"=w81:T5[])  [unwired: 6 in]
      }
      event "Intensity Time Trace": Shortcut Menu Activation? {
        n42 = event-data() -> ("CtlRef"=w95:refnum<vi>, "MenuRef"=w94:refnum<k9>)  [unwired: 1 in]
        n43 = call "XY Graph Check-Uncheck Menu Items.vi"("Menu in"=w94, "XY Graph Refnum"=w95) -> ("Error Out (dup)"=w96:errorcluster, "Menu out"=w101:refnum<k9>, "XY Graph Refnum dup"=w103:T11)  [unwired: 6 in, 1 out]
        n44 = call "XY Graph Get Label.vi"("XYGraph"=w103) -> ("Graph Label"=w104:string)  [unwired: 8 in]
        n45 = case shown="\"\", Default" w104 {
          tunnel: w96 -> [w105 w111]
          tunnel: [w105 w110] -> w100
          tunnel: w101 -> [w106 w109]
          tunnel: [w106 w108] -> w102
          frame "", Default {
          }
          frame "Decay Graph" {
            n46 = call "AlliGator Decay Graph Get-Set Process Plot Target.vi"("Get (F)/Set"=FALSE, "Error In"=w111, "Menu"=w109) -> ("Error Out (dup)"=w110:errorcluster, "Menu"=w108:refnum<k9>)  [unwired: 6 in, 1 out]
          }
        }
        n47 = call "AlliGator Add Python Functions to Object Menu.vi"("error in (no error)"=w100, "Menu in"=w102, "Object Refnum"=w103) -> ("error out"=w97:errorcluster, "Menu out"=w98:refnum<k9>, "Object Refnum dup"=w99:refnum<vi>)  [unwired: 6 in]
        n48 = call "AlliGator Grayed out Menu Items.vi"("error in (no error)"=w97, "Menu in"=w98, "Object Refnum"=w99) -> ("error out"=w93:errorcluster)  [unwired: 7 in, 1 out]
        n49 = event-data() -> ()  [unwired: 2 in, 1 out]
      }
      event "Time Step": Value Change {
        n50 = event-data() -> ("CtlRef"=w120:refnum<vi>)  [unwired: 1 in]
        n51 = property class="DigNum (strict)"(reference=w120) -> (reference out=w121:refnum<vi>, error out=w122:errorcluster, "Label.Text"=w118:string, "Value"=w117:dbl[unit])  [unwired: 1 in]
        n52 = call "AlliGator Update Settings & Control.vi"("Error In"=w122, "Value"=w117, "Sender"=w119, "CtlRef"=w121) -> ("Error Out"=w113:errorcluster)  [unwired: 7 in]
        n53 = node(w117) -> (w114:dbl)
        n54 = property on="Intensity Time Trace" class="XYGraph (strict)"(error in=w113, "XScale.Multiplier"=w114) -> (error out=w112:errorcluster)  [unwired: 1 in, 1 out]
        n55 = call "AlliGator Get Control Notebook String.vi"("error in (no error)"=w112, "Value"=w117, "Control Label"=w118) -> ("error out"=w115:errorcluster, "Notebook String"=w116:string)  [unwired: 7 in]
      }
      event "Use File Timestamp": Value Change {
        n56 = event-data() -> ("CtlRef"=w128:refnum<vi>, "OldVal"=w127:bool, "NewVal"=w126:bool)  [unwired: 1 in]
        n57 = case shown="True" w125 {
          tunnel: w126 -> [_ w133]
          tunnel: w128 -> [w131 _]
          tunnel: w127 -> [w130 _]
          tunnel: [w129 _] -> w123
          tunnel: [_ w132] -> w124
          frame False {
            n58 = property class="Bool (strict)"(reference=w131, "Value"=w130) -> (error out=w129:errorcluster)  [unwired: 1 in, 1 out]
          }
          frame True {
            n59 = Bundle By Name(cluster=T5 {"AlliGator Q Event"=enum."Intensity Time Trace:Use File Timestamp", "Data"=variant} ("element"), "Data"=w133) -> (w134:T5)
            n60 = Build Array(w134) -> (w132:T5[])
          }
        }
      }
      event "Use Intensity Correction File": Value Change {
        n61 = event-data() -> ("NewVal"=w141:bool, "CtlRef"=w142:refnum<vi>, "OldVal"=w143:bool)  [unwired: 1 in]
        n62 = case shown="True" w139 {
          tunnel: w140 -> [_ w156]
          tunnel: w142 -> [w146 w154]
          tunnel: w141 -> [_ w152]
          tunnel: w143 -> [w145 _]
          tunnel: [w144 w155] -> w136
          tunnel: [_ w149] -> w138
          tunnel: [_ w148] -> w137
          frame False {
            n63 = property class="Bool (strict)"(reference=w146, "Value"=w145) -> (error out=w144:errorcluster)  [unwired: 1 in, 1 out]
          }
          frame True {
            n64 = local read "Intensity Correction File"() -> (w147:path)
            n65 = property class="Bool (strict)"(reference=w154) -> (reference out=w158:refnum<vi>, error out=w151:errorcluster, "Label.Text"=w159:string, "Value"=w157:bool)  [unwired: 1 in]
            n66 = Empty String/Path?(string/path=w147) -> (empty?=w160:bool)
            n67 = Compound Arithmetic op=AND(w152, invert w160) -> (w153:bool)
            n68 = case shown="True" w153 {
              tunnel: w147 -> [_ w162]
              tunnel: [_ w161] -> w149
              frame False {
              }
              frame True {
                n69 = Bundle By Name(cluster=T5 {"AlliGator Q Event"=enum."Intensity Time Trace:Load Intensity Corrections File", "Data"=variant} ("Time-Gated Phasor Q Element"), "Data"=w162) -> (w163:T5)
                n70 = Build Array(w163) -> (w161:T5[])
              }
            }
            n71 = call "AlliGator Update Settings & Control.vi"("Error In"=w151, "Value"=w157, "Sender"=w156, "CtlRef"=w158) -> ("Error Out"=w150:errorcluster)  [unwired: 7 in]
            n72 = call "AlliGator Get Control Notebook String.vi"("error in (no error)"=w150, "Value"=w157, "Control Label"=w159) -> ("error out"=w155:errorcluster, "Notebook String"=w148:string)  [unwired: 7 in]
          }
        }
      }
      event User Event {
        n73 = event-data() -> ("subpanel"=w167:string, "event"=w166:string)  [unwired: 1 in]
        n74 = case shown="\"AlliGator\"" w167 {
          tunnel: w166 -> [_ w169]
          tunnel: [_ w168] -> w165
          frame "False", Default {
          }
          frame "AlliGator" {
            n75 = case shown="\"quit\"" w169 {
              tunnel: [_ TRUE] -> w168
              frame "False", Default {
              }
              frame "quit" {
              }
            }
          }
        }
      }
      event Mouse Enter {
        n76 = event-data() -> ("CtlRef"=w172:refnum<vi>)  [unwired: 1 in]
        n77 = Unbundle By Name(w173) -> ("Event Registration Refnum"=w175:refnum<event-registration>)
        n78 = call "XY Graph Tipstrip Mouse Enter.vi"("Event Registration Refnum"=w175, "XY Graph Refnum"=w172) -> ("Event Registration Refnum"=w174:refnum<event-registration>)  [unwired: 8 in, 1 out]
        n79 = Bundle By Name(cluster=w173, "Event Registration Refnum"=w174) -> (w171:T3)
      }
      event Mouse Leave {
        n80 = event-data() -> ("CtlRef"=w177:refnum<vi>)  [unwired: 1 in]
        n81 = Unbundle By Name(w178) -> ("Event Registration Refnum"=w179:refnum<event-registration>)
        n82 = call "XY Graph Tipstrip Mouse Leave.vi"("Event Registration Refnum"=w179, "XY Graph Refnum"=w177) -> ("Event Registration Refnum"=w180:refnum<event-registration>)  [unwired: 8 in, 1 out]
        n83 = Bundle By Name(cluster=w178, "Event Registration Refnum"=w180) -> (w176:T3)
      }
      event Mouse Move {
        n84 = event-data() -> ("CtlRef"=w183:refnum<vi>, "Coords"=w182:T8)  [unwired: 1 in]
        n85 = control-ref of="Intensity Time Trace TipStrip"() -> (w181:refnum<vi>)
        n86 = call "XY Graph Set Plot TipStrip.vi"("TipStrip Refnum"=w181, "Max Length (200)"=300, "Coords"=w182, "XY Graph Refnum"=w183) -> ()  [unwired: 5 in, 3 out]
      }
    }
    n87 = call "AlliGator Settings Storage.vi"("AlliGator Settings List"=AlliGator_Settings_List."Miscellaneous:Verbose Error Mode") -> ("Variant Data out"=w46:variant)  [unwired: 9 in, 1 out]
    n88 = call-poly "Variant to Data.vi"("Variant"=w46) -> ("Value"=w39:bool)  [unwired: 8 in]
    n89 = call "Send Message to Notebook.vi"("Error In"=w41, "Text"=w38, "Notebook Queue"=w40) -> ("Error Out"=w43:errorcluster, "Notebook Queue"=w42:refnum<queue>)  [unwired: 5 in]
    n90 = call "Light Theme Message Style.vi"() -> ()  [unwired: 1 out]
    n91 = call "AlliGator Queue Non Empty Events.vi"("Actions"=w36, "AlliGator Q"=w37) -> ()  [unwired: 9 in, 1 out]
    n92 = call "Send Error to Notebook.vi"("error in (no error)"=w43, "Verbose Error Messages (T)"=w39, "State Machine Case Error Source"="Intensity Time Trace", "Notebook Q"=w42) -> ("Error Out"=w30:errorcluster)  [unwired: 7 in]
  }
  n93 = call "Tiny Clear Error.vi"("Error In"=w23) -> ("no Error Out"=w22:errorcluster)  [unwired: 8 in]
  n94 = Unregister For Events(event registration refnum=w24) -> (error out=w14:errorcluster)  [unwired: 1 in]
  n95 = invoke class="VI" method="FP.Close"(reference=w5, error in=w22) -> (error out=w15:errorcluster)  [unwired: 1 in, 2 out]
  n96 = Merge Errors(w15, w14) -> (w13:errorcluster)
  n97 = call "Tiny Clear Error.vi"("Error In"=w13) -> ()  [unwired: 8 in, 1 out]
